vi "Status Tree to JSON.vi"(4 "Status Tree":map{string[], T1}(c390)) -> (7 "JSON":string)   [LabVIEW 2020, in "Volatus.lvlib" / "DebugHTTPController.lvclass"]
uses:
  DebugHTTPController.lvclass
  Module Status.ctl
  Module/State.ctl
  lv-cdm/CDM-Config/Config-JSON/Config-JSON.lvclass
  lv-cdm/CDM-Config/Config Element/Write Variant Value.vi
  DebugHTTPController.lvclass/DebugHTTPController.ctl
  lv-cdm/CDM-Config/Config Manager/Config Manager.lvclass
  lv-cdm/CDM-Config/Config Element/Config Element.lvclass
  Module/Module.lvclass
  Volatus.lvlib
panel:
  out "error out":errorcluster
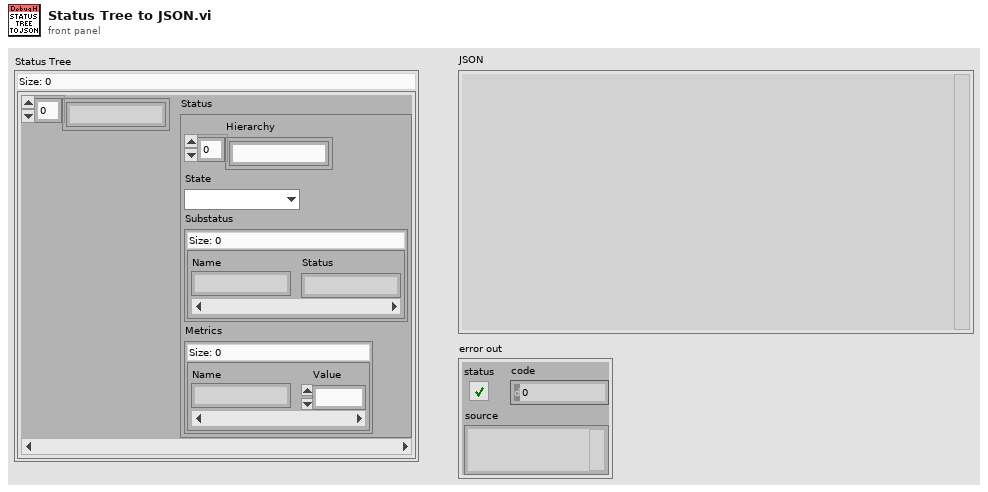
[diagram p1: front panel]
types:
  T1 = typedef "Volatus.lvlib/Module Status.ctl" = cluster{"Hierarchy":string[], "State":T2, "Substatus":map{string, string}, "Metrics":map{string, dbl}}
  T2 = typedef "Volatus.lvlib/Module.lvclass/State.ctl" = enum16{"Unknown", "Launched", "Starting", "Running", "Stopping", "Stopped", "Error - Starting", "Error - Run", "Error - Stopping"}
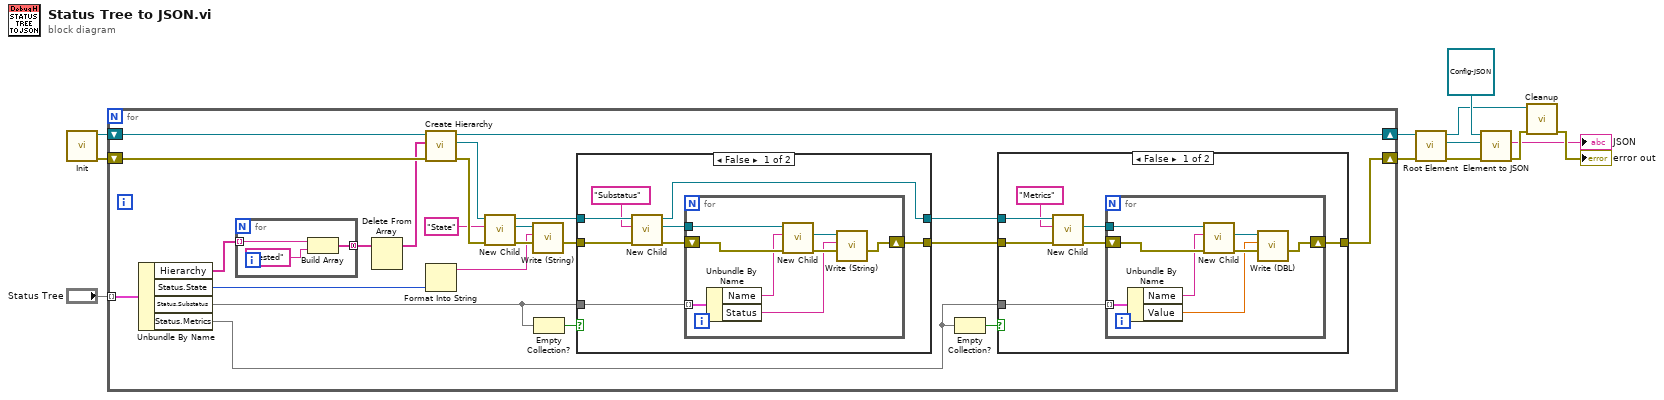
[diagram p0: block diagram]
diagram:
  n1 = call "Init.vi"() -> ("error out"=w8:errorcluster, "Config Manager out"=w10:refnum<class "Config Manager.lvclass">)  [unwired: 10 in]
  n2 = for {
    shift-right: [w30] -> w7
    shift-left: w10 -> [w32]
    tunnel: "Status Tree" -> [w33] mode=indexing
    shift-right: [w13] -> w6
    shift-left: w8 -> [w34]
    n3 = Unbundle By Name(w33) -> ("Hierarchy"=w29:string[], "Status.State"=w31:T2, "Status.Substatus"=w21:map{string, string}, "Status.Metrics"=w16:map{string, dbl})
    n4 = for {
      tunnel: w29 -> [w72] mode=indexing
      tunnel: [w70] -> w28 mode=concatenating
      n5 = Build Array(w72, "Nested" ("element")) -> (w70:string[])
    }
    n6 = Delete From Array(array=w28) -> (array with subset deleted=w27:string[])  [unwired: 2 in, 1 out]
    n7 = call "Create Hierarchy.vi"("error in (no error)"=w34, "Hierarchy"=w27, "Config Manager in"=w32) -> ("error out"=w35:errorcluster, "Leaf Element"=w26:refnum<class "Config Element.lvclass">, "Config Manager out"=w30:refnum<class "Config Manager.lvclass">)  [unwired: 6 in]
    n8 = Format Into String(w31) -> (resulting string=w22:string)  [unwired: 3 in, 1 out]
    n9 = call "New Child.vi"("error in (no error)"=w35, "Child Name"="State", "Config Element in"=w26) -> ("error out"=w24:errorcluster, "New Child"=w23:refnum<class "Config Element.lvclass">, "Config Element out"=w19:refnum<class "Config Element.lvclass">)  [unwired: 6 in]
    n10 = call "Write (String).vi"("error in (no error)"=w24, "String Value"=w22, "Config Element in"=w23) -> ("error out"=w18:errorcluster)  [unwired: 7 in, 1 out]
    n11 = Empty Collection?(1:w21) -> (0:w20:bool)
    n12 = case shown="False" w20 {
      tunnel: w21 -> [w54 _]
      tunnel: w19 -> [w58 w68]
      tunnel: w18 -> [w59 w69]
      tunnel: [w53 w69] -> w14
      tunnel: [w52 w68] -> w15
      frame False {
        n13 = call "New Child.vi"("error in (no error)"=w59, "Child Name"="Substatus", "Config Element in"=w58) -> ("error out"=w56:errorcluster, "New Child"=w55:refnum<class "Config Element.lvclass">, "Config Element out"=w52:refnum<class "Config Element.lvclass">)  [unwired: 6 in]
        n14 = for {
          shift-right: [w61] -> w53
          shift-left: w56 -> [w67]
          tunnel: w55 -> [w65]
          tunnel: w54 -> [w66] mode=indexing
          n15 = Unbundle By Name(w66) -> ("Name"=w64:string, "Status"=w60:string)
          n16 = call "New Child.vi"("error in (no error)"=w67, "Child Name"=w64, "Config Element in"=w65) -> ("error out"=w63:errorcluster, "New Child"=w62:refnum<class "Config Element.lvclass">)  [unwired: 6 in, 1 out]
          n17 = call "Write (String).vi"("error in (no error)"=w63, "String Value"=w60, "Config Element in"=w62) -> ("error out"=w61:errorcluster)  [unwired: 7 in, 1 out]
        }
      }
      frame True {
      }
    }
    n18 = Empty Collection?(1:w16) -> (0:w17:bool)
    n19 = case shown="False" w17 {
      tunnel: w16 -> [w37 _]
      tunnel: w15 -> [w41 _]
      tunnel: w14 -> [w42 w51]
      tunnel: [w36 w51] -> w13
      frame False {
        n20 = call "New Child.vi"("error in (no error)"=w42, "Child Name"="Metrics", "Config Element in"=w41) -> ("error out"=w39:errorcluster, "New Child"=w38:refnum<class "Config Element.lvclass">)  [unwired: 6 in, 1 out]
        n21 = for {
          shift-right: [w44] -> w36
          shift-left: w39 -> [w50]
          tunnel: w38 -> [w48]
          tunnel: w37 -> [w49] mode=indexing
          n22 = Unbundle By Name(w49) -> ("Name"=w47:string, "Value"=w43:dbl)
          n23 = call "New Child.vi"("error in (no error)"=w50, "Child Name"=w47, "Config Element in"=w48) -> ("error out"=w46:errorcluster, "New Child"=w45:refnum<class "Config Element.lvclass">)  [unwired: 6 in, 1 out]
          n24 = call "Write (DBL).vi"("error in (no error)"=w46, "DBL Value"=w43, "Config Element in"=w45) -> ("error out"=w44:errorcluster)  [unwired: 7 in, 1 out]
        }
      }
      frame True {
      }
    }
  }
  n25 = call "Root Element.vi"("error in (no error)"=w6, "Config Manager in"=w7) -> ("error out"=w4:errorcluster, "Root Element"=w5:refnum<class "Config Element.lvclass">, "Config Manager out"=w1:refnum<class "Config Manager.lvclass">)  [unwired: 7 in]
  n26 = call "Element to JSON.vi"("error in (no error)"=w4, "Element"=w5, "Config-JSON"=refnum<class "Config-JSON.lvclass"> refnum) -> ("error out"=w12:errorcluster, "JSON"=→"JSON":string)  [unwired: 7 in]
  n27 = call "Cleanup.vi"("error in (no error)"=w12, "Config Manager in"=w1) -> ("error out"=→"error out":errorcluster)  [unwired: 9 in]
